vi "Robot Main.vi"() -> ()   [LabVIEW 2023]
panel:
  in  "Logging Config":T1={"Enable"=FALSE, "Log Path"=path "", "Log Flush (s)"=0.25}
  # "Enable and configure on-robot logging\nof NT writes (lossless). Files are given\nsuffix of .wpilog and saved in \n/home/systemcore/logs/."
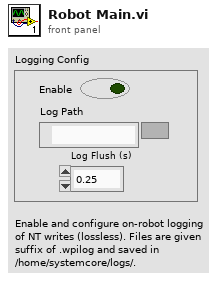
[diagram p1: front panel]
types:
  T1 = cluster{"Enable":bool, "Log Path":path, "Log Flush (s)":dbl}
  T2 = typedef "DS OpModes.ctl" = cluster{"Autos":refnum<vi>[], "Teles":refnum<vi>[], "Utilities":refnum<vi>[]}
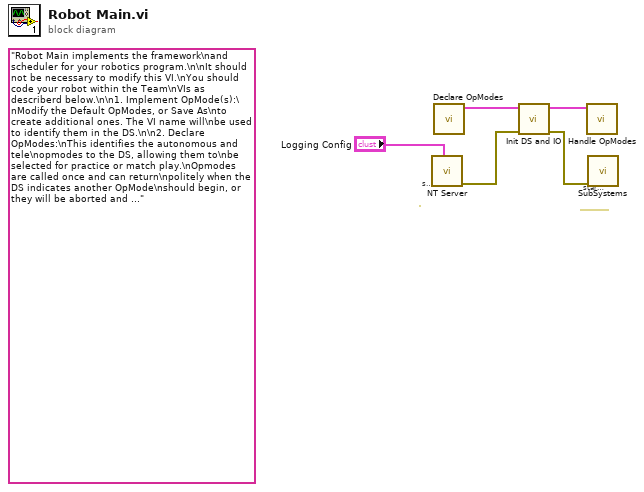
[diagram p0: block diagram]
diagram:
  (unwired) "Robot Main implements the framework\nand scheduler for your robotics program.\n\nIt should not be necessary to modify this VI.\nYou should code your robot within the Team\nVIs as describerd below.\n\n1. Implement OpMode(s):\nModify the Default OpModes, or Save As\nto create additional ones. The VI name will\nbe used to identify them in the DS.\n\n2. Declare OpModes:\nThis identifies the autonomous and tele\nopmodes to the DS, allowing them to\nbe selected for practice or match play.\nOpmodes are called once and can return\npolitely when the DS indicates another OpMode\nshould begin, or they will be aborted and the\nnew OpMode started.\n\n3. OpModes can directly control I/O or\nthey can command subSystems which\ncontrol the I/O. To add subSystems, right-\nclick on the project and New >> SubSystem. "
  # "start subSystems"
  # "start NT"
  n1 = call <vilib>:"NT Server.vi"("Logging Config"="Logging Config") -> ("error out"=w1:errorcluster)  [unwired: 10 in]
  n2 = call "Declare OpModes.vi"() -> ("OpModes"=w4:T2)  [unwired: 11 in]
  n3 = call <vilib>:"Init DS and IO.vi"("error in"=w1, "OpModes"=w4) -> ("error out"=w2:errorcluster, "OpModes"=w3:T2)  [unwired: 8 in]
  n4 = call <vilib>:"Handle OpModes.vi"("OpModes"=w3) -> ()  [unwired: 11 in]
  n5 = call "SubSystems.vi"("error in (no error)"=w2) -> ()  [unwired: 11 in]
